vi "VIH Project Tree - Get Project Files & Groups (Ext).vi"(8 "error in":errorcluster, 10 "Parent Item Tag (Root)":string, 11 "Project Tree":T1) -> (0 "error out":errorcluster, 1 "Project Files":T3, 3 "dup Project Tree":T1, 4 "Project Group IDs":string[](array[string]))   [LabVIEW 2014]
doc: "::: VI Helpeks :::\nCopyright (c) 2000-2026 Konstantin Shifershteyn. All rights reserved."
uses:
  VIH Project Tree Typedef - Tree Refnum.ctl
  _VIH HelpGen - Palette.llb/VIH HelpGen Typedef - Palette - Item Type Enum.ctl
panel:
  # "VI Helpeks\nCopyright (c) 2012-2026 Konstantin Shifershteyn"
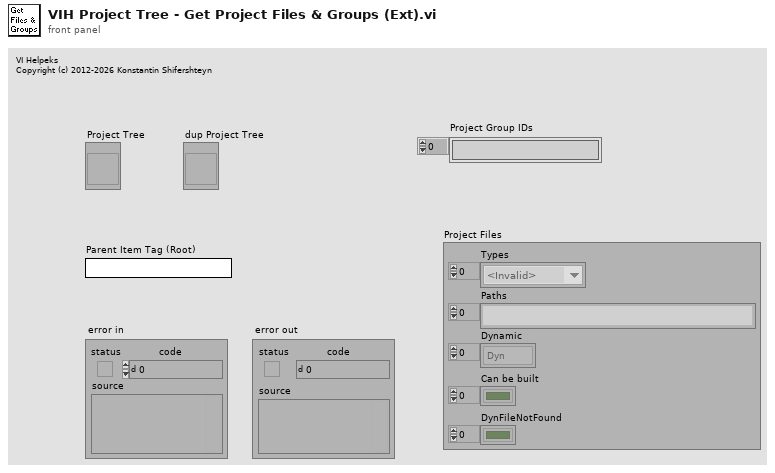
[diagram p1: front panel]
types:
  T1 = typedef "VIH Project Tree Typedef - Tree Refnum.ctl" = refnum<vi>
  T2 = typedef "VIH HelpGen Typedef - Palette - Item Type Enum.ctl" = enum32{"<Invalid>", "<unknown>", "VI", "Menu", "LV Func", "Express VI", "Poly VI", "CTL", "HTML"}
  T3 = cluster{"Types":T2[], "Paths":path[], "Dynamic":enum16{"Dyn", "Stat", "Both"}[], "Can be built":bool[], "DynFileNotFound":bool[]}
  T4 = cluster{"Types":T2[], "Paths":path[], "Dynamic":enum16{"Dyn", "Stat", "Both"}[], "Can be built":bool[], "NotFound":bool[]}
  T5 = typedef "VIH Project Tree Typedef - Tree Item Type.ctl" = enum32{"<Invalid>", "Project", "Proj Files", "Proj Rules", "File Group", "Rule Group", "Any File", "LV Func", ".mnu", ".mnu (dyn)", ".vi", ".vi (dyn)", ".vit", ".vit (dyn)", ".ctl", ".ctl (dyn)", ".ctt", ".ctt (dyn)", "polyVI", "polyVI (dyn)", "expVI", "expVI (dyn)", "HTML", "PolyVI Inst"}
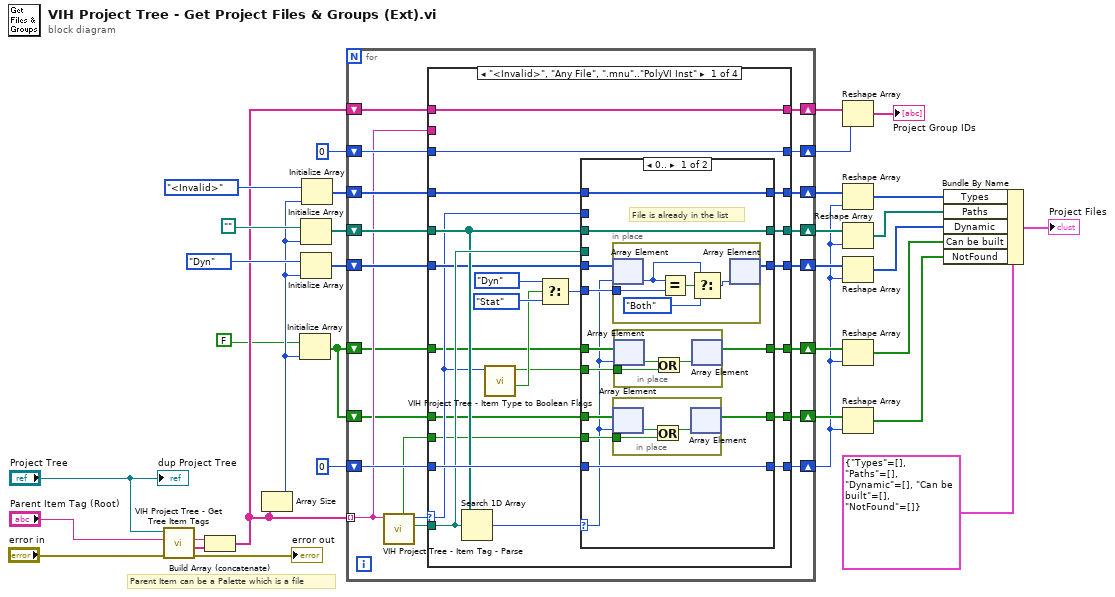
[diagram p0: block diagram]
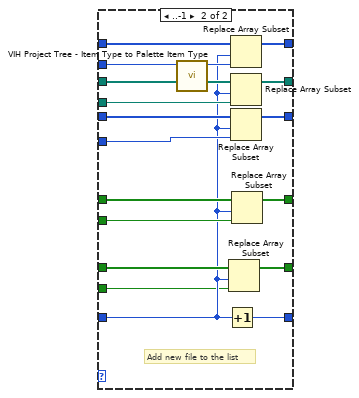
[diagram p2: hidden frame]
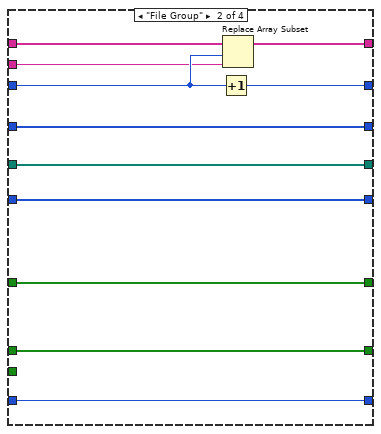
[diagram p3: hidden frame]
diagram:
  # "Parent Item can be a Palette which is a file"
  n1 = call "VIH Project Tree - Get Tree Item Tags.vi"("error in"="error in", "Parent Item Tag"="Parent Item Tag (Root)", "Project Tree"="Project Tree") -> ("error out"=→"error out":errorcluster, "Child Item Tags"=w17:string[], "dup Parent Item Tag"=w16:string)  [unwired: 5 in, 1 out]
  n2 = Build Array (concatenate)(w16, w17) -> (w15:string[])
  n3 = Array Size(array=w15) -> (size(s)=w8:i32)
  n4 = Initialize Array(FALSE, w8) -> (w4:bool[])
  n5 = Initialize Array(path "", w8) -> (w24:path[])
  n6 = Initialize Array(enum16{"Dyn", "Stat", "Both"}."Dyn", w8) -> (w33:enum16{"Dyn", "Stat", "Both"}[])
  n7 = Initialize Array(VIH_HelpGen_Typedef_-_Palette_-_Item_Type_Enum."<Invalid>" ("Item/File Type"), w8) -> (w23:T2[])
  n8 = for {
    tunnel: w15 -> [w40] mode=indexing
    shift-right: [w49] -> w27
    shift-left: w23 -> [w53]
    shift-right: [w48] -> w26
    shift-left: w24 -> [w52]
    shift-right: [w47] -> w2
    shift-left: 0 -> [w51]
    shift-right: [w45] -> w31
    shift-left: w33 -> [w46]
    shift-right: [w44] -> w13
    shift-left: w15 -> [w43]
    shift-right: [w42] -> w12
    shift-left: 0 -> [w41]
    shift-right: [w38] -> w6
    shift-left: w4 -> [w39]
    shift-right: [w36] -> w3
    shift-left: w4 -> [w37]
    n9 = call "VIH Project Tree - Item Tag - Parse.vi"("Tree Item Tag"=w40) -> ("Item File Path"=w50:path, "Item Type"=w54:T5, "Not Found"=w35:bool)  [unwired: 8 in]
    n10 = case shown="\"<Invalid>\", \"Any File\", \".mnu\"..\"PolyVI Inst\"" w54 {
      selector: w54 -> [w62 _ _ _]
      tunnel: w53 -> [w77 w130 w138 w146]
      tunnel: w52 -> [w71 w129 w137 w145]
      tunnel: w51 -> [w74 w128 w136 w144]
      tunnel: w50 -> [w72 _ _ _]
      tunnel: [w76 w130 w138 w146] -> w49
      tunnel: [w75 w129 w137 w145] -> w48
      tunnel: [w73 w128 w136 w144] -> w47
      tunnel: w46 -> [w70 w127 w135 w143]
      tunnel: [w69 w127 w135 w143] -> w45
      tunnel: [w64 w125 w134 w142] -> w44
      tunnel: w43 -> [w64 w126 w134 w142]
      tunnel: [w63 w123 w133 w141] -> w42
      tunnel: w41 -> [w63 w124 w133 w141]
      tunnel: w40 -> [_ w122 _ _]
      tunnel: w39 -> [w60 w121 w132 w140]
      tunnel: [w59 w121 w132 w140] -> w38
      tunnel: w37 -> [w57 w120 w131 w139]
      tunnel: [w56 w120 w131 w139] -> w36
      tunnel: w35 -> [w55 _ _ _]
      frame "<Invalid>", "Any File", ".mnu".."PolyVI Inst" {
        n11 = Search 1D Array(1D array=w71, element=w72) -> (index of element=w68:i32)  [unwired: 1 in]
        n12 = call "VIH Project Tree - Item Type to Boolean Flags.vi"("Item Type"=w62) -> ("Dynamic"=w61:bool, "Can be built"=w58:bool)  [unwired: 4 in, 5 out]
        n13 = Select(t=enum16{"Dyn", "Stat", "Both"}."Dyn", s=w61, f=enum16{"Dyn", "Stat", "Both"}."Stat") -> (s? t:f=w65:enum16{"Dyn", "Stat", "Both"})
        n14 = case shown="0.." w68 {
          selector: w68 -> [w78 _]
          tunnel: w77 -> [w90 w119]
          tunnel: w62 -> [_ w114]
          tunnel: [w90 w118] -> w76
          tunnel: [w89 w117] -> w75
          tunnel: w74 -> [w88 w103]
          tunnel: [w88 w116] -> w73
          tunnel: w72 -> [_ w109]
          tunnel: w71 -> [w89 w115]
          tunnel: w70 -> [w87 w112]
          tunnel: [w86 w111] -> w69
          tunnel: w65 -> [w85 w110]
          tunnel: w60 -> [w83 w108]
          tunnel: [w82 w107] -> w59
          tunnel: w58 -> [w84 w106]
          tunnel: w57 -> [w81 w105]
          tunnel: [w80 w104] -> w56
          tunnel: w55 -> [w79 w102]
          frame 0.. {
            # "File is already in the list"
            n15 = in-place {
              in-place-border: w85 -> [w98]
              n16 = in-place-array #1(w87, w78) -> (w99:enum16{"Dyn", "Stat", "Both"})
              n17 = Equal?(x=w99, y=w98) -> (x = y?=w101:bool)
              n18 = Select(t=w99, s=w101, f=enum16{"Dyn", "Stat", "Both"}."Both" ("y")) -> (s? t:f=w100:enum16{"Dyn", "Stat", "Both"})
              n19 = in-place-array #1(w100) -> (w86:enum16{"Dyn", "Stat", "Both"}[])  [unwired: 1 out]
            }
            n20 = in-place {
              in-place-border: w79 -> [w92]
              n21 = in-place-array #2(w81, w78) -> (w93:bool)
              n22 = Or(x=w93, y=w92) -> (x .or. y?=w91:bool)
              n23 = in-place-array #2(w91) -> (w80:bool[])  [unwired: 1 out]
            }
            n24 = in-place {
              in-place-border: w84 -> [w95]
              n25 = in-place-array #3(w83, w78) -> (w96:bool)
              n26 = Or(x=w96, y=w95) -> (x .or. y?=w94:bool)
              n27 = in-place-array #3(w94) -> (w82:bool[])  [unwired: 1 out]
            }
          }
          frame ..-1 {
            # "Add new file to the list"
            n28 = call "VIH Project Tree - Item Type to Palette Item Type.vi"("Tree Item Type"=w114) -> ("Item/File Type"=w113:T2)  [unwired: 9 in, 1 out]
            n29 = Increment(x=w103) -> (x+1=w116:i32)
            n30 = Replace Array Subset(array=w105, new element=w102, index=w103) -> (w104:bool[])
            n31 = Replace Array Subset(array=w119, new element=w113, index=w103) -> (w118:T2[])
            n32 = Replace Array Subset(array=w115, new element=w109, index=w103) -> (w117:path[])
            n33 = Replace Array Subset(array=w112, new element=w110, index=w103) -> (w111:enum16{"Dyn", "Stat", "Both"}[])
            n34 = Replace Array Subset(array=w108, new element=w106, index=w103) -> (w107:bool[])
          }
        }
      }
      frame "File Group" {
        n35 = Increment(x=w124) -> (x+1=w123:i32)
        n36 = Replace Array Subset(array=w126, new element=w122, index=w124) -> (w125:string[])
      }
      frame "Project".."Proj Rules", "Rule Group" {
      }
      frame "LV Func" {
      }
    }
  }
  n37 = Reshape Array(w13, w12) -> (→"Project Group IDs":string[])
  n38 = Reshape Array(w27, w2) -> (w28:T2[])
  n39 = Reshape Array(w26, w2) -> (w29:path[])
  n40 = Reshape Array(w31, w2) -> (w32:enum16{"Dyn", "Stat", "Both"}[])
  n41 = Reshape Array(w6, w2) -> (w5:bool[])
  n42 = Reshape Array(w3, w2) -> (w1:bool[])
  n43 = Bundle By Name(cluster=T4 {"Types"=[], "Paths"=[], "Dynamic"=[], "Can be built"=[], "NotFound"=[]} ("Project Files"), "Types"=w28, "Paths"=w29, "Dynamic"=w32, "Can be built"=w5, "NotFound"=w1) -> (→"Project Files":T4)
  "dup Project Tree" <- "Project Tree"
